vi "test_GetItemInfosFromProjectFile_SplitProjectTargetsSolution.vi"() -> (3 "Pass?":bool)   [LabVIEW 2019, in "Tests.SolutionBuilder.lvlib"]
uses:
  Tests.SolutionBuilder.lvlib
  SolutionBuilder/SolutionBuilder.lvclass
  SolutionBuilder/ProjectItem/ProjectItem.lvclass
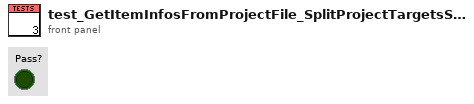
[diagram p1: front panel]
types:
  T1 = typedef "SolutionBuilder.lvlib/SolutionBuilder.lvclass/ProjectItemMap.ctl" = map{path, refnum<class "ProjectItem.lvclass">[]}
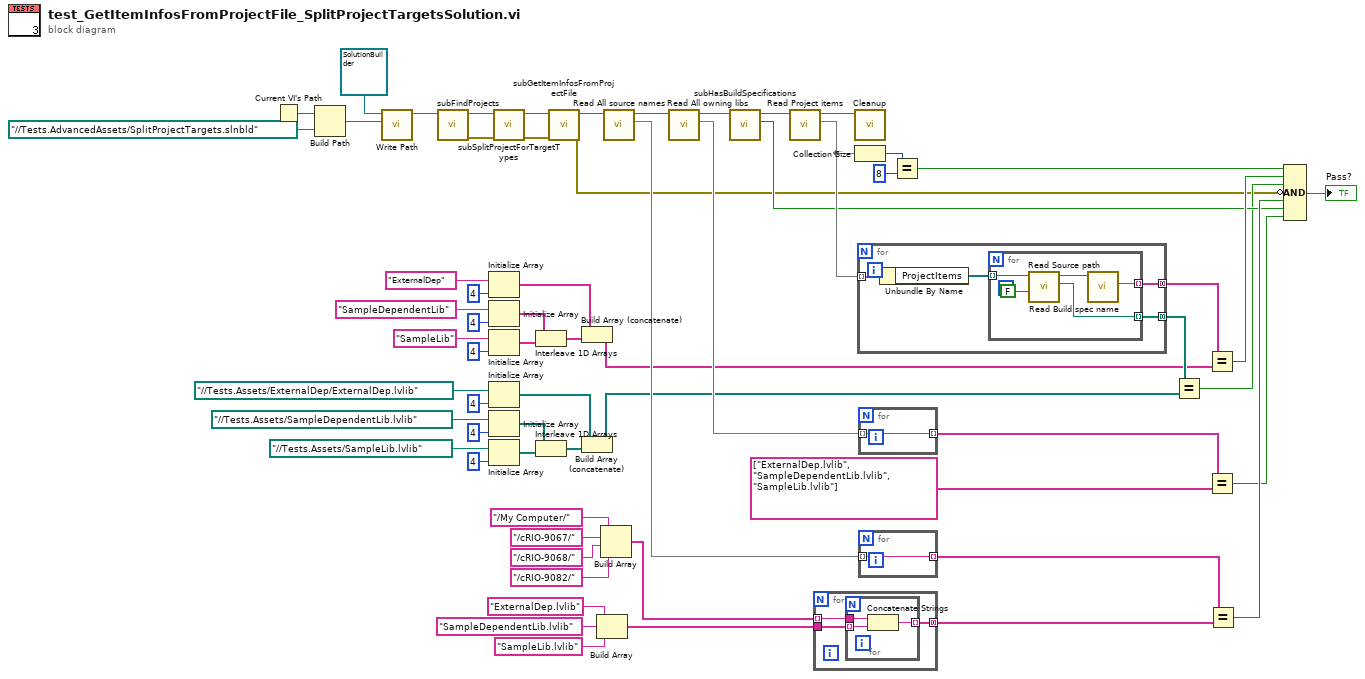
[diagram p0: block diagram]
diagram:
  n1 = Current VI's Path() -> (path=w63:path)
  n2 = Build Path(base path=w63, name or relative path=path "../../Tests.AdvancedAssets/SplitProjectTargets.slnbld" ("Path")) -> (appended path=w61:path)
  n3 = call "Write Path.vi"("Path"=w61, "SolutionBuilder in"=refnum<class "SolutionBuilder.lvclass"> refnum) -> ("SolutionBuilder out"=w1:refnum<class "SolutionBuilder.lvclass">)  [unwired: 9 in]
  n4 = call "subFindProjects.vi"("SolutionBuilder in"=w1) -> ("error out"=w5:errorcluster, "SolutionBuilder out"=w4:refnum<class "SolutionBuilder.lvclass">)  [unwired: 9 in]
  n5 = Initialize Array("ExternalDep" ("Build spec name"), 4 ("dimension size")) -> (w30:string[])
  n6 = Initialize Array("SampleDependentLib" ("Build spec name"), 4 ("dimension size")) -> (w33:string[])
  n7 = Initialize Array("SampleLib" ("Build spec name"), 4 ("dimension size")) -> (w32:string[])
  n8 = Initialize Array(path "../../Tests.Assets/ExternalDep/ExternalDep.lvlib" ("Source path"), 4 ("dimension size")) -> (w28:path[])
  n9 = Initialize Array(path "../../Tests.Assets/SampleDependentLib.lvlib" ("Source path"), 4 ("dimension size")) -> (w25:path[])
  n10 = Initialize Array(path "../../Tests.Assets/SampleLib.lvlib" ("Source path"), 4 ("dimension size")) -> (w26:path[])
  n11 = call "subSplitProjectForTargetTypes.vi"("error in (no error)"=w5, "SolutionBuilder in"=w4) -> ("error out"=w2:errorcluster, "SolutionBuilder out"=w3:refnum<class "SolutionBuilder.lvclass">)  [unwired: 8 in]
  n12 = Interleave 1D Arrays(w33, w32) -> (w31:string[])
  n13 = Interleave 1D Arrays(w25, w26) -> (w27:path[])
  n14 = call "subGetItemInfosFromProjectFile.vi"("error in (no error)"=w2, "SolutionBuilder in"=w3) -> ("error out"=w40:errorcluster, "SolutionBuilder out"=w58:refnum<class "SolutionBuilder.lvclass">)  [unwired: 8 in]
  n15 = Build Array (concatenate)(w30, w31) -> (w29:string[])
  n16 = Build Array (concatenate)(w28, w27) -> (w18:path[])
  n17 = Build Array("ExternalDep.lvlib" ("Build spec name"), "SampleDependentLib.lvlib" ("Build spec name"), "SampleLib.lvlib" ("Build spec name")) -> (w9:string[])
  n18 = Build Array("/My Computer/" ("Build spec name"), "/cRIO-9067/" ("Build spec name"), "/cRIO-9068/" ("Build spec name"), "/cRIO-9082/" ("Build spec name")) -> (w10:string[])
  n19 = call "Read All source names.vi"("SolutionBuilder in"=w58) -> ("All source names"=w54:set{string}, "SolutionBuilder out"=w46:refnum<class "SolutionBuilder.lvclass">)  [unwired: 9 in]
  n20 = call "Read All owning libs.vi"("SolutionBuilder in"=w46) -> ("All owning libs"=w44:set{string}, "SolutionBuilder out"=w45:refnum<class "SolutionBuilder.lvclass">)  [unwired: 9 in]
  n21 = call "subHasBuildSpecifications.vi"("SolutionBuilder in"=w45) -> ("Has specs?"=w51:bool, "SolutionBuilder out"=w52:refnum<class "SolutionBuilder.lvclass">)  [unwired: 8 in, 1 out]
  n22 = call "Read Project items.vi"("SolutionBuilder in"=w52) -> ("Project items"=w57:T1, "SolutionBuilder out"=w6:refnum<class "SolutionBuilder.lvclass">)  [unwired: 9 in]
  n23 = for {
    tunnel: w10 -> [w67] mode=indexing
    tunnel: w9 -> [w66]
    tunnel: [w65] -> w8 mode=concatenating
    n24 = for {
      tunnel: w67 -> [w70]
      tunnel: w66 -> [w69] mode=indexing
      tunnel: [w68] -> w65 mode=indexing
      n25 = Concatenate Strings(w70, w69) -> (w68:string)
    }
  }
  n26 = call "Cleanup.vi"("SolutionBuilder in"=w6) -> ()  [unwired: 9 in, 2 out]
  n27 = Collection Size(1:w57) -> (0:w60:i32)
  n28 = for {
    tunnel: w57 -> [w74] mode=indexing
    tunnel: [w73] -> w50 mode=concatenating
    tunnel: [w71] -> w48 mode=concatenating
    n29 = Unbundle By Name(w74) -> ("ProjectItems"=w72:refnum<class "ProjectItem.lvclass">[])
    n30 = for {
      tunnel: w72 -> [w77] mode=indexing
      tunnel: [w79] -> w73 mode=indexing
      tunnel: [w76] -> w71 mode=indexing
      n31 = call "Read Source path.vi"("Force abs path? (T)"=FALSE, "ProjectItem in"=w77) -> ("Source path"=w76:path, "ProjectItem out"=w78:refnum<class "ProjectItem.lvclass">)  [unwired: 8 in]
      n32 = call "Read Build spec name.vi"("ProjectItem in"=w78) -> ("Build spec name"=w79:string)  [unwired: 9 in, 1 out]
    }
  }
  n33 = for {
    tunnel: w44 -> [w80] mode=indexing
    tunnel: [w80] -> w43 mode=indexing
  }
  n34 = for {
    tunnel: w54 -> [w81] mode=indexing
    tunnel: [w81] -> w49 mode=indexing
  }
  n35 = Equal?(x=w60, y=8) -> (x = y?=w56:bool)
  n36 = Equal?(x=w48, y=w18) -> (x = y?=w47:bool)
  n37 = Equal?(x=w50, y=w29) -> (x = y?=w55:bool)
  n38 = Equal?(x=w43, y=string[] ["ExternalDep.lvlib", "SampleDependentLib.lvlib", "SampleLib.lvlib"] ("Array")) -> (x = y?=w41:bool)
  n39 = Equal?(x=w49, y=w8) -> (x = y?=w53:bool)
  n40 = Compound Arithmetic op=AND(w56, w55, w47, invert w40, w53, w51, w41) -> (→"Pass?":bool)
